vi "IsValidNode.vi"(10 "Node Name":string, 11 "Server in":refnum<class "Server.lvclass">) -> (2 "Valid Node Definition?":bool, 3 "Server out":refnum<class "Server.lvclass">)   [LabVIEW 2020, in "jki_python_bridge.lvlib" / "Server.lvclass"]
uses:
  Server.lvclass
  Server.lvclass/Server.ctl
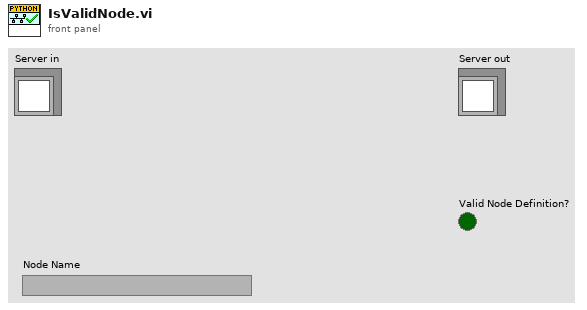
[diagram p1: front panel]
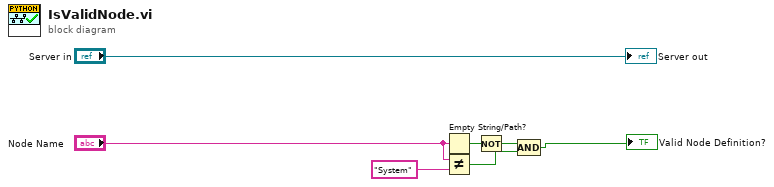
[diagram p0: block diagram]
diagram:
  n1 = Empty String/Path?(string/path="Node Name") -> (empty?=w4:bool)
  n2 = Not Equal?(x="Node Name", y="System") -> (x != y?=w1:bool)
  n3 = Not(x=w4) -> (.not. x?=w3:bool)
  n4 = Compound Arithmetic op=AND(w3, w1) -> (→"Valid Node Definition?":bool)
  "Server out" <- "Server in"
